vi "lab3_1.vi"() -> ()   [LabVIEW 2025]
uses:
  <vilib>/eio/EIONode/EIONode.xnode
  <vilib>/rvi/DataTransferAndStorage/Container/XNode/niFpgaContainer.xnode
  <vilib>/rvi/interface/RandomDataEmulation/nirviRandomDataFpgaReadWriteTemplate.vi
  <vilib>/rvi/eio/common/nirviEmuTemplateMethod_errors.vi
panel:
  in  "Treshold":i16
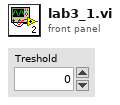
[diagram p1: front panel]
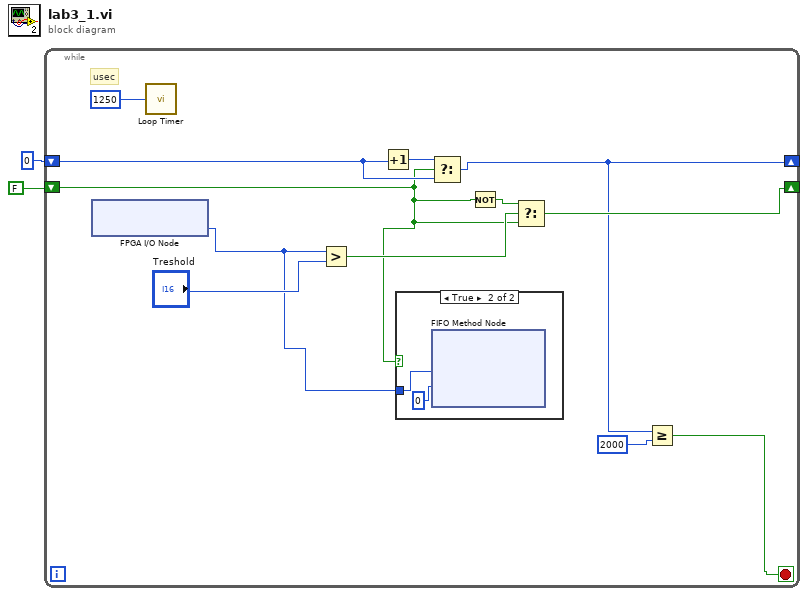
[diagram p0: block diagram]
diagram:
  n1 = while {
    shift-right: [w7] -> _
    shift-left: i16 0 -> [w11]
    shift-right: [w8] -> _
    shift-left: FALSE -> [w3]
    stop <- w5 stop-if-true
    # "usec"
    n2 = xnode "FPGA I/O Node"() -> ("AccelerationX"=w4:i16)  [unwired: 1 in, 1 out]
    n3 = call "Loop Timer"("Count(uSec)"=u32 1250) -> ()  [unwired: 1 out]
    n4 = Greater?(x=w4, y="Treshold") -> (0:w10:bool)
    n5 = Increment(x=w11) -> (x+1=w12:i16)
    n6 = case shown="True" w3 {
      tunnel: w4 -> [_ w16]
      frame False {
      }
      frame True {
        n7 = xnode ("FIFO Method Node")("Element"=w16, "Timeout"=0) -> ()  [unwired: 1 in, 2 out]
      }
    }
    n8 = Select(t=w12, s=w3, f=w11) -> (s? t:f=w7:i16)
    n9 = Not(x=w3) -> (.not. x?=w9:bool)
    n10 = Select(t=w9, s=w10, f=w3) -> (s? t:f=w8:bool)
    n11 = Greater Or Equal?(x=w7, y=i16 2000) -> (x >= y?=w5:bool)
  }
